vi "Read Batch Values - Variant.vi"(8 "error in (no error)":errorcluster, 11 "OD Batch in":refnum<class "OD Batch.lvclass">) -> (0 "error out":errorcluster, 2 "Array":cluster{"Variant":variant, "type":T1}[](array[cluster]), 3 "OD Batch out":refnum<class "OD Batch.lvclass">)   [LabVIEW 2023, in "xnet_canopen.lvlib" / "OD Batch.lvclass"]
uses:
  OD Batch.lvclass
  OD Batch.lvclass/OD Batch.ctl
  Read Batch OD By Array Index - bool.vi
  Read Batch OD By Array Index - i8.vi
  Read Batch OD By Array Index - i16.vi
  Read Batch OD By Array Index - i32.vi
  Read Batch OD By Array Index - u8.vi
  Read Batch OD By Array Index - u16.vi
  Read Batch OD By Array Index - u32.vi
  Read Batch OD By Array Index - f32.vi
  Read Batch OD By Array Index - string.vi
  Read Batch OD By Array Index - bytes.vi
  Read Batch OD By Array Index - f64.vi
  Read Batch OD By Array Index - i64.vi
  Read Batch OD By Array Index - u64.vi
  <vilib>/Utility/Data Type/NI_Data Type.lvlib
  <vilib>/Utility/Data Type/Type Definitions/Data Type.ctl
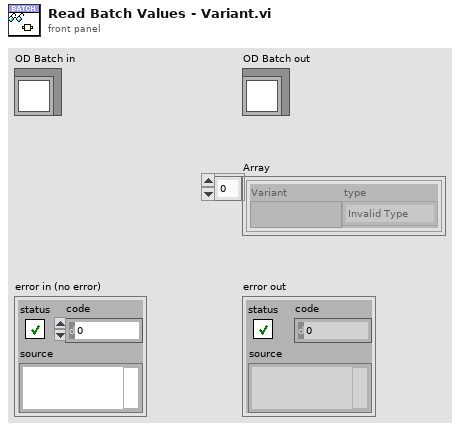
[diagram p1: front panel]
types:
  T1 = typedef "NI_Data Type.lvlib/Data Type.ctl" = enum8{"Invalid Type", "Void", "I8", "I16", "I32", "I64", "U8", "U16", "U32", "U64", "Single Float", "Double Float", "Extended Float", "Single Complex", "Double Complex", "Extended Complex", "Enum U8", "Enum U16", "Enum U32", "Enum U64", "Single Float With Unit", "Double Float With Unit", "Extended Float With Unit", "Single Complex with Unit", "Double Complex with Unit", "Extended Complex with Unit", "Boolean", "String", "Path", "Picture", "Tag", "Array", "Cluster", "Variant", "LV Variant", "Waveform", "Timestamp", "Digital Waveform", "Digital Data", "ExpressData", "Refnum", "External Data", "VI", "Poly VI", "LabVIEW Class Instance", "Fixed Point", "Set Collection", "Map Collection"}
  T2 = typedef "xnet_canopen.lvlib/od entry.ctl" = cluster{"OD Index":T3, "CANOpen Types":T4, "Size":u32, "Offset":u32, "Value":variant, "Initialized":bool}
  T3 = typedef "xnet_canopen.lvlib/od index.ctl" = cluster{"Index":u16, "SubIndex":u8}
  T4 = typedef "xnet_canopen.lvlib/canopen types.ctl" = u32
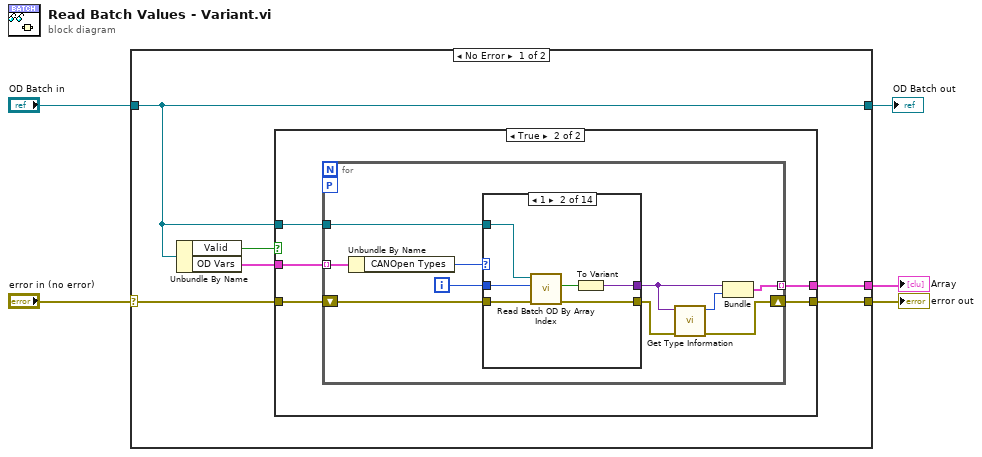
[diagram p0: block diagram]
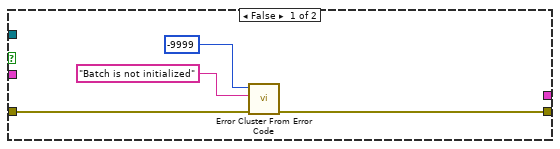
[diagram p2: hidden frame]
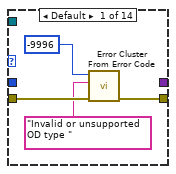
[diagram p3: hidden frame]
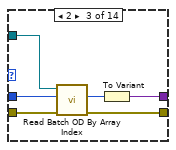
[diagram p4: hidden frame]
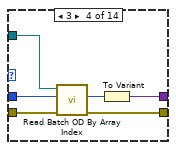
[diagram p5: hidden frame]
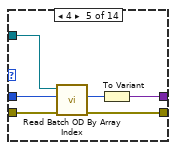
[diagram p6: hidden frame]
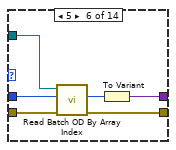
[diagram p7: hidden frame]
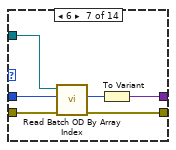
[diagram p8: hidden frame]
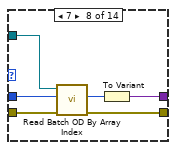
[diagram p9: hidden frame]
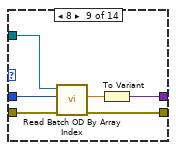
[diagram p10: hidden frame]
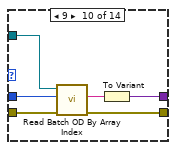
[diagram p11: hidden frame]
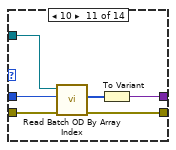
[diagram p12: hidden frame]
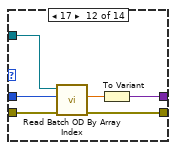
[diagram p13: hidden frame]
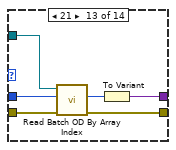
[diagram p14: hidden frame]
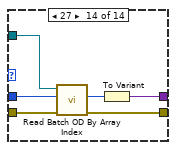
[diagram p15: hidden frame]
diagram:
  n1 = case shown="No Error" "error in (no error)" {
    selector: "error in (no error)" -> [w11 w113]
    tunnel: [w10 w113] -> w4
    tunnel: [w8 w114] -> w2
    tunnel: "OD Batch in" -> [w8 w114]
    tunnel: [w7 _] -> w1
    frame No Error {
      n2 = Unbundle By Name(w8) -> ("Valid"=w6:bool, "OD Vars"=w9:T2[])
      n3 = case shown="True" w6 {
        tunnel: w11 -> [w13 w20]
        tunnel: [w12 w19] -> w10
        tunnel: w9 -> [_ w18]
        tunnel: w8 -> [_ w17]
        tunnel: [_ w16] -> w7
        frame False {
          n4 = call <vilib>:"Error Cluster From Error Code.vi"("error in (no error)"=w13, "error message (\"\")"="Batch is not initialized" ("error message (\"\")"), "error code (0)"=-9999) -> ("error out"=w12:errorcluster)  [unwired: 6 in]
        }
        frame True {
          n5 = for {
            shift-right: [w23] -> w19
            shift-left: w20 -> [w30]
            tunnel: w18 -> [w28] mode=indexing
            workers-P: _ -> [_]
            tunnel: w17 -> [w25]
            tunnel: [w24] -> w16 mode=indexing
            i -> [w26]
            n6 = Unbundle By Name(w28) -> ("CANOpen Types"=w27:T4)
            n7 = case shown="1" w27 {
              tunnel: w30 -> [w34 w40 w46 w52 w58 w64 w70 w76 w82 w88 w94 w100 w106 w112]
              tunnel: [w33 w39 w45 w51 w57 w63 w69 w75 w81 w87 w93 w99 w105 w111] -> w29
              tunnel: w26 -> [_ w38 w44 w50 w56 w62 w68 w74 w80 w86 w92 w98 w104 w110]
              tunnel: w25 -> [_ w37 w43 w49 w55 w61 w67 w73 w79 w85 w91 w97 w103 w109]
              tunnel: [_ w35 w41 w47 w53 w59 w65 w71 w77 w83 w89 w95 w101 w107] -> w21
              frame Default {
                n8 = call <vilib>:"Error Cluster From Error Code.vi"("error in (no error)"=w34, "error message (\"\")"="Invalid or unsupported OD type " ("error message (\"\")"), "error code (0)"=-9996) -> ("error out"=w33:errorcluster)  [unwired: 6 in]
              }
              frame 1 {
                n9 = call-poly "Read Batch OD By Array Index.vi"("error in (no error)"=w40, "array index"=w38, "OD Batch in"=w37) -> ("error out"=w39:errorcluster, "value"=w36:bool)  [unwired: 6 in, 1 out]
                n10 = To Variant(anything=w36) -> (Variant=w35:variant)
              }
              frame 2 {
                n11 = call-poly "Read Batch OD By Array Index.vi"("error in (no error)"=w46, "array index"=w44, "OD Batch in"=w43) -> ("error out"=w45:errorcluster, "value"=w42:i8)  [unwired: 6 in, 1 out]
                n12 = To Variant(anything=w42) -> (Variant=w41:variant)
              }
              frame 3 {
                n13 = call-poly "Read Batch OD By Array Index.vi"("error in (no error)"=w52, "array index"=w50, "OD Batch in"=w49) -> ("error out"=w51:errorcluster, "value"=w48:i16)  [unwired: 6 in, 1 out]
                n14 = To Variant(anything=w48) -> (Variant=w47:variant)
              }
              frame 4 {
                n15 = call-poly "Read Batch OD By Array Index.vi"("error in (no error)"=w58, "array index"=w56, "OD Batch in"=w55) -> ("error out"=w57:errorcluster, "value"=w54:i32)  [unwired: 6 in, 1 out]
                n16 = To Variant(anything=w54) -> (Variant=w53:variant)
              }
              frame 5 {
                n17 = call-poly "Read Batch OD By Array Index.vi"("error in (no error)"=w64, "array index"=w62, "OD Batch in"=w61) -> ("error out"=w63:errorcluster, "value"=w60:u8)  [unwired: 6 in, 1 out]
                n18 = To Variant(anything=w60) -> (Variant=w59:variant)
              }
              frame 6 {
                n19 = call-poly "Read Batch OD By Array Index.vi"("error in (no error)"=w70, "array index"=w68, "OD Batch in"=w67) -> ("error out"=w69:errorcluster, "value"=w66:u16)  [unwired: 6 in, 1 out]
                n20 = To Variant(anything=w66) -> (Variant=w65:variant)
              }
              frame 7 {
                n21 = call-poly "Read Batch OD By Array Index.vi"("error in (no error)"=w76, "array index"=w74, "OD Batch in"=w73) -> ("error out"=w75:errorcluster, "value"=w72:u32)  [unwired: 6 in, 1 out]
                n22 = To Variant(anything=w72) -> (Variant=w71:variant)
              }
              frame 8 {
                n23 = call-poly "Read Batch OD By Array Index.vi"("error in (no error)"=w82, "array index"=w80, "OD Batch in"=w79) -> ("error out"=w81:errorcluster, "value"=w78:sgl)  [unwired: 6 in, 1 out]
                n24 = To Variant(anything=w78) -> (Variant=w77:variant)
              }
              frame 9 {
                n25 = call-poly "Read Batch OD By Array Index.vi"("error in (no error)"=w88, "array index"=w86, "OD Batch in"=w85) -> ("error out"=w87:errorcluster, "value"=w84:string)  [unwired: 6 in, 1 out]
                n26 = To Variant(anything=w84) -> (Variant=w83:variant)
              }
              frame 10 {
                n27 = call-poly "Read Batch OD By Array Index.vi"("error in (no error)"=w94, "array index"=w92, "OD Batch in"=w91) -> ("error out"=w93:errorcluster, "value"=w90:u8[])  [unwired: 6 in, 1 out]
                n28 = To Variant(anything=w90) -> (Variant=w89:variant)
              }
              frame 17 {
                n29 = call-poly "Read Batch OD By Array Index.vi"("error in (no error)"=w100, "array index"=w98, "OD Batch in"=w97) -> ("error out"=w99:errorcluster, "value"=w96:dbl)  [unwired: 6 in, 1 out]
                n30 = To Variant(anything=w96) -> (Variant=w95:variant)
              }
              frame 21 {
                n31 = call-poly "Read Batch OD By Array Index.vi"("error in (no error)"=w106, "array index"=w104, "OD Batch in"=w103) -> ("error out"=w105:errorcluster, "value"=w102:i64)  [unwired: 6 in, 1 out]
                n32 = To Variant(anything=w102) -> (Variant=w101:variant)
              }
              frame 27 {
                n33 = call-poly "Read Batch OD By Array Index.vi"("error in (no error)"=w112, "array index"=w110, "OD Batch in"=w109) -> ("error out"=w111:errorcluster, "value"=w108:u64)  [unwired: 6 in, 1 out]
                n34 = To Variant(anything=w108) -> (Variant=w107:variant)
              }
            }
            n35 = call <vilib>:"Get Type Information.vi"("error in (no error)"=w29, "variant"=w21) -> ("error out"=w23:errorcluster, "type"=w22:T1)  [unwired: 5 in, 3 out]
            n36 = Bundle("Variant"=w21, "type"=w22) -> (w24:cluster{"Variant":variant, "type":T1})  [unwired: 1 in]
          }
        }
      }
    }
    frame Error {
    }
  }
  "error out" <- w4
  "OD Batch out" <- w2
  "Array" <- w1
